vi "SubscribeHeaterStateUpdated Finish Stream.vi"(11 "Stream Data in":T1={"gRPCid"=0, "Active"=FALSE, "timeout"=-1}) -> (0 "error out":errorcluster)   [LabVIEW 2020]
doc: "Send dummy message with the <b>Streaming?</b> parameter set to False to singal stop of stream."
uses:
  Stream Data--cluster.ctl
  <vilib>/gRPC/LabVIEW gRPC Library/Shared/grpcId.ctl
  thermal-chamber-controller_server/RPC Messages/lv_python_grpc_webui_demo_v1_HeaterStateUpdated.ctl
  thermal-chamber-controller_server/RPC Messages/lv_python_grpc_webui_demo_v1_HeaterState.ctl
  thermal-chamber-controller_server/thermal-chamber-controller_server.lvlib
  thermal-chamber-controller_server/RPC Service/ThermalChamberController/ThermalChamberController.lvclass
  <vilib>/gRPC/LabVIEW gRPC Library/grpc-lvsupport-release.lvlib
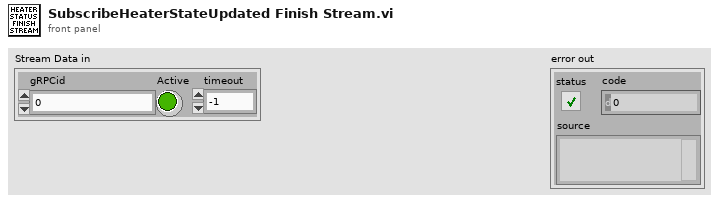
[diagram p1: front panel]
types:
  T1 = typedef "Stream Data--cluster.ctl" = cluster{"gRPCid":T2, "Active":bool, "timeout":i32}
  T2 = typedef "grpc-lvsupport-release.lvlib/grpcId.ctl" = u64
  T3 = typedef "thermal-chamber-controller_server.lvlib/lv_python_grpc_webui_demo_v1_HeaterStateUpdated.ctl" = cluster{"heater_state":T4}
  T4 = typedef "thermal-chamber-controller_server.lvlib/lv_python_grpc_webui_demo_v1_HeaterState.ctl" = enum32{"HEATER_ENABLED", "HEATER_DISABLED"}
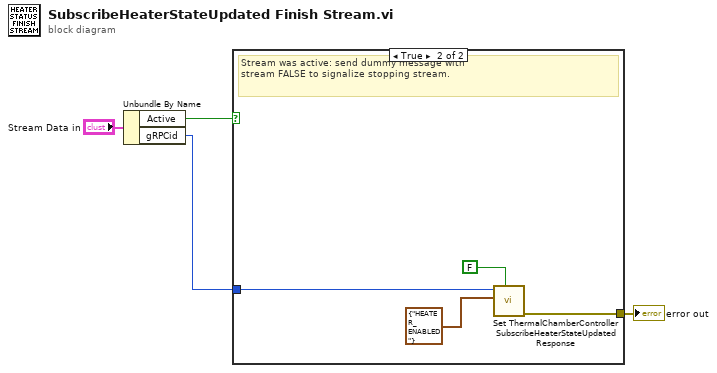
[diagram p0: block diagram]
diagram:
  n1 = Unbundle By Name("Stream Data in") -> ("Active"=w4:bool, "gRPCid"=w3:T2)
  n2 = case shown="True" w4 {
    tunnel: w3 -> [_ w8]
    tunnel: [_ w6] -> w1
    frame False {
      # "Stream was not active."
    }
    frame True {
      # "Stream was active: send dummy message with \nstream FALSE to signalize stopping stream."
      n3 = call "Set ThermalChamberController SubscribeHeaterStateUpdated Response.vi"("Streaming? (F)"=FALSE, "Message Data"=T3 {"heater_state"=enum."HEATER_ENABLED"}, "gRPCid in"=w8) -> ("error out"=w6:errorcluster)  [unwired: 8 in]
    }
  }
  "error out" <- w1
